vi "Build and Parse.vi"() -> ()   [LabVIEW 2021]
uses:
  <vilib>/xnet/xnet.llb/XNET Frame CAN.ctl
  <vilib>/xnet/xnet.llb/XNET Frame Type CAN.ctl
  XNET CAN RW.lvclass
  C:/Program Files/National Instruments/LabVIEW 2021/vi.lib/CIF Foundation/CIF CAN RW Core/CAN_RW_CORE.lvclass
  <vilib>/CIF Foundation/CIF CAN RW Core/CAN_RW_CORE.lvclass/CAN_RW_CORE.ctl
  <vilib>/CIF Foundation/CIF PCAP Parse and Build/pcap_Parse_Build_CIF.lvclass/pcap_Parse_Build_CIF.ctl
  Utilities/XNET CAN to Header Cluster.vi
  <vilib>/CIF Foundation/CIF PCAP Parse and Build/Build/Build Packet Header.vi
  <vilib>/CIF Foundation/CIF PCAP Parse and Build/Build/SubVIs/Flatten SocketCAN Header.vi
  <vilib>/CIF Foundation/CIF CAN RW Core/Utilities/Filter Packets.vi
  <vilib>/CIF Foundation/CIF CAN RW Core/Accessors/Read CAN Interface Mode.vi
  <vilib>/CIF Foundation/CIF CAN RW Core/Accessors/Read pcap class.vi
  Utilities/Header Cluster to XNET CAN.vi
  <vilib>/CIF Foundation/CIF PCAP Parse and Build/Parse/Parse Packet Header.vi
  <vilib>/CIF Foundation/CIF PCAP Parse and Build/Parse/Unflatten Socket CAN Header.vi
  <vilib>/CIF Foundation/CIF PCAP Parse and Build/Utilities/Get Data Segment.vi
  <vilib>/CIF Foundation/CIF PCAP Parse and Build/Data Accessors/Read Offset.vi
  <vilib>/CIF Foundation/CIF CAN RW Core/Accessors/Write pcap class.vi
  <vilib>/CIF Foundation/CIF PCAP Parse and Build/Data Accessors/Write Offset.vi
  <vilib>/CIF Foundation/CIF Utilities/Time/System Time/LabVIEW Time to TAI Time.vi
  <vilib>/CIF Foundation/CIF PCAP Parse and Build/Build/SubVIs/Flatten Packet Header.vi
  <vilib>/CIF Foundation/CIF Utilities/DataTypes/Flatten Unflatten/Flatten U32.vi
  <vilib>/CIF Foundation/CIF Utilities/Time/System Time/TAI Time to LabVIEW Time.vi
  <vilib>/CIF Foundation/CIF PCAP Parse and Build/Parse/Unflatten Packet Header.vi
  <vilib>/CIF Foundation/CIF Utilities/DataTypes/Flatten Unflatten/Unflatten U32.vi
  <vilib>/CIF Foundation/CIF PCAP Parse and Build/Utilities/Add Error.vi
  <vilib>/CIF Foundation/CIF Utilities/Errors/Append Error Location.vi
  <vilib>/CIF Foundation/CIF PCAP Parse and Build/pcap_Parse_Build_CIF.lvclass
panel:
  out "error out":errorcluster
  out "Local Subordinate":T1[](array[typedef])=[{"timestamp"=timestamp(3831573600 s since 1904-01-01), "payload"=[0, 0, 0, 0, 0, 0, 0, 4], "identifier"=83, "type"=16, "extended?"=TRUE, "echo?"=FALSE}, {"timestamp"=timestamp(2082844800 s since 1904-01-01), "payload"=[0, 0, 0, 0, 0, 0, 0, 4], "identifier"=50, "type"=8, "extended?"=FALSE, "echo?"=FALSE}] {"payload" format="%x"; "timestamp" format="%<%.7X\n%x>T"; "type" items=["CAN Data"=0, "CAN Remote"=1, "CAN Bus Error"=2, "CAN 2.0 Data"=8, "CAN FD Data"=16, "CAN FD+BRS Data"=24, "J1939 Data"=192, "Delay"=224, "Log Trigger"=225, "Start Trigger"=226]; "identifier" format="%x"}
  in  "XNET CAN Data":T1[](array[typedef])=[{"timestamp"=timestamp(3831573600 s since 1904-01-01), "payload"=[0, 0, 0, 0, 0, 0, 0, 4], "identifier"=83, "type"=16, "extended?"=TRUE, "echo?"=FALSE}, {"timestamp"=timestamp(0 s since 1904-01-01), "payload"=[0, 0, 0, 0, 0, 0, 0, 4], "identifier"=50, "type"=0, "extended?"=FALSE, "echo?"=FALSE}] {"payload" format="%x"; "timestamp" format="%<%.7X\n%x>T"; "type" items=["CAN Data"=0, "CAN Remote"=1, "CAN Bus Error"=2, "CAN 2.0 Data"=8, "CAN FD Data"=16, "CAN FD+BRS Data"=24, "J1939 Data"=192, "Delay"=224, "Log Trigger"=225, "Start Trigger"=226]; "identifier" format="%x"}
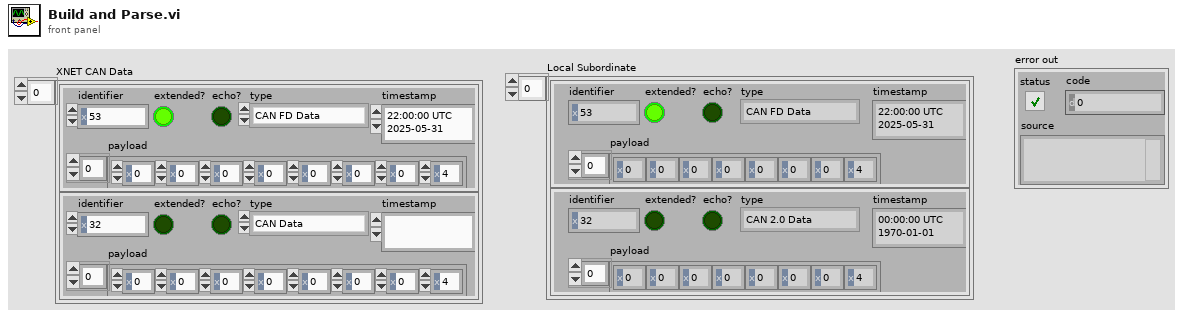
[diagram p1: front panel]
types:
  T1 = typedef "XNET Frame CAN.ctl" = cluster{"timestamp":timestamp, "payload":u8[], "identifier":u32, "type":T2, "extended?":bool, "echo?":bool}
  T2 = typedef "XNET Frame Type CAN.ctl" = u8
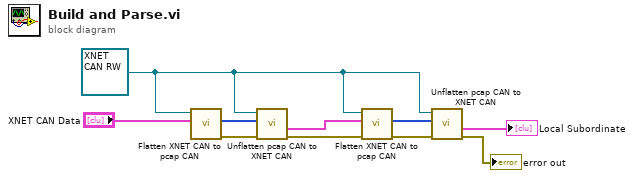
[diagram p0: block diagram]
diagram:
  w4 = refnum<class "XNET CAN RW.lvclass"> refnum ("XNET_CAN_RW in")
  n1 = call "Flatten XNET CAN to pcap CAN.vi"("XNET CAN Data"="XNET CAN Data", "XNET_CAN_RW in"=w4) -> ("error out"=w3:errorcluster, "pcap CAN DATA"=w7:u8[])  [unwired: 7 in, 1 out]
  n2 = call "Unflatten pcap CAN to XNET CAN.vi"("error in (no error)"=w3, "pcap CAN DATA in"=w7, "XNET_CAN_RW in"=w4) -> ("error out"=w2:errorcluster, "XNET CAN Data"=w6:T1[])  [unwired: 3 in, 4 out]
  n3 = call "Flatten XNET CAN to pcap CAN.vi"("error in (no error)"=w2, "XNET CAN Data"=w6, "XNET_CAN_RW in"=w4) -> ("error out"=w1:errorcluster, "pcap CAN DATA"=w5:u8[])  [unwired: 6 in, 1 out]
  n4 = call "Unflatten pcap CAN to XNET CAN.vi"("error in (no error)"=w1, "pcap CAN DATA in"=w5, "XNET_CAN_RW in"=w4) -> ("error out"=→"error out":errorcluster, "XNET CAN Data"=→"Local Subordinate":T1[])  [unwired: 3 in, 4 out]
